vi "Get TestSuite Test Paths__core.vi"(8 "error in (no error)":errorcluster, 11 "Test Project":path) -> (0 "error out":errorcluster, 2 "Test Paths":path[](array[path]))   [LabVIEW 2013, in "GraphicalTestRunner.lvlib"]
uses:
  GraphicalTestRunner.lvlib
  Classes/TestLoader/TestLoader.lvclass
  Classes/TestSuite/TestSuite.lvclass
  <userlib>/_OpenG.lib/array/array.llb/Remove Duplicates from 1D Array (Path)__ogtk.vi
  JKI Reuse/Is an Error (error cluster)__jki_lib_error_handling -- VI Tester.vi
  Libraries/VITesterUtilities.lvlib
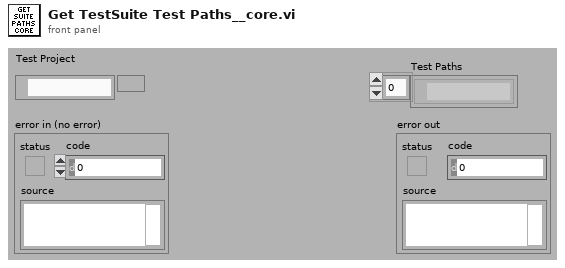
[diagram p1: front panel]
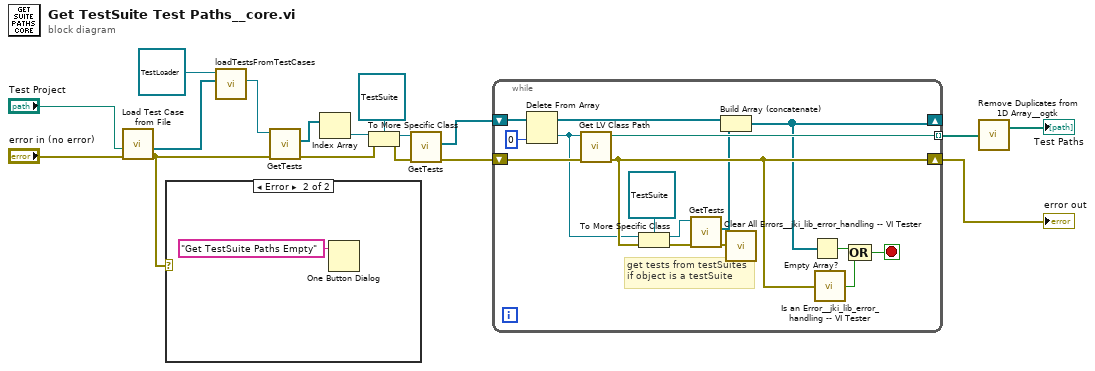
[diagram p0: block diagram]
diagram:
  n1 = call "Load Test Case from File.vi"("error in"="error in (no error)", "Test Class Path"="Test Project") -> ("error out"=w1:errorcluster, "Test Case"=w3:refnum<class>[])  [unwired: 8 in]
  n2 = case shown="Error" w1 {
    frame No Error {
    }
    frame Error {
      n3 = One Button Dialog(message="Get TestSuite Paths Empty") -> ()  [unwired: 1 in, 1 out]
    }
  }
  n4 = call-dynamic "loadTestsFromTestCases.vi"("Tests"=w3, "TestLoader in"=refnum<class "TestLoader.lvclass"> refnum ("reference in")) -> ("TestSuite"=w4:refnum<class "TestSuite.lvclass">)  [unwired: 7 in, 2 out]
  n5 = call-dynamic "GetTests.vi"("error in (no error)"=w1, "TestSuite in"=w4) -> ("error out"=w10:errorcluster, "tests"=w5:refnum<class>[])  [unwired: 7 in, 1 out]
  n6 = Index Array(array=w5) -> (element=w6:refnum<class>)  [unwired: 1 in]
  n7 = To More Specific Class(target class=refnum<class "TestSuite.lvclass"> refnum ("TestSuite"), reference=w6, error in=w10) -> (specific class reference=w9:refnum<class "TestSuite.lvclass">, error out=w8:errorcluster)
  n8 = call-dynamic "GetTests.vi"("error in (no error)"=w8, "TestSuite in"=w9) -> ("error out"=w13:errorcluster, "tests"=w11:refnum<class>[])  [unwired: 7 in, 1 out]
  n9 = while {
    tunnel: [w34] -> w12 mode=indexing
    shift-right: [w23] -> w14
    shift-left: w13 -> [w33]
    shift-right: [w21] -> _
    shift-left: w11 -> [w32]
    stop <- w27 stop-if-true
    # "get tests from testSuites\nif object is a testSuite"
    n10 = Delete From Array(array=w32, index=0) -> (deleted portion=w22:refnum<class>, array with subset deleted=w30:refnum<class>[])  [unwired: 1 in]
    n11 = call <vilib>:"Get LV Class Path.vi"("error in (no error)"=w33, "object"=w22) -> ("error out"=w23:errorcluster, "class path"=w34:path)  [unwired: 8 in]
    n12 = To More Specific Class(target class=refnum<class "TestSuite.lvclass"> refnum ("TestSuite"), reference=w22, error in=w23) -> (specific class reference=w24:refnum<class "TestSuite.lvclass">, error out=w25:errorcluster)
    n13 = call-dynamic "GetTests.vi"("error in (no error)"=w25, "TestSuite in"=w24) -> ("error out"=w19:errorcluster, "tests"=w20:refnum<class>[])  [unwired: 7 in, 1 out]
    n14 = Build Array (concatenate)(w30, w20) -> (w21:refnum<class>[])
    n15 = call "Clear All Errors__jki_lib_error_handling -- VI Tester.vi"("error in"=w19) -> ()  [unwired: 4 in, 1 out]
    n16 = Empty Array?(array=w21) -> (empty?=w29:bool)
    n17 = call-poly "Is an Error__jki_lib_error_handling -- VI Tester.vi"("error in"=w23) -> ("error?"=w28:bool)  [unwired: 8 in]
    n18 = Compound Arithmetic op=OR(w29, w28) -> (w27:bool)
  }
  "error out" <- w14
  n19 = call-poly <userlib>:"Remove Duplicates from 1D Array__ogtk.vi"("Input Array"=w12) -> ("Output Array"=→"Test Paths":path[])  [unwired: 1 out]
